vi "Update Device ID.vi"(8 "error in (no error)":errorcluster caption="에러 입력(에러 없음)", 11 "Instrument Manager 입력":refnum<class "Instrument Manager.lvclass">) -> (0 "error out":errorcluster caption="에러 출력", 3 "Instrument Manager 출력":refnum<class "Instrument Manager.lvclass">)   [LabVIEW 2023, in "Instrument Manager.lvclass"]
uses:
  Instrument Manager.lvclass
  Instrument Manager.lvclass/Instrument Manager.ctl
  Module/Turn Table and Mast Control/Class/CO3000/CO3000.lvclass
  Module/Turn Table and Mast Control/Interface Class/Turn Table/Interface - Turn Table.lvclass
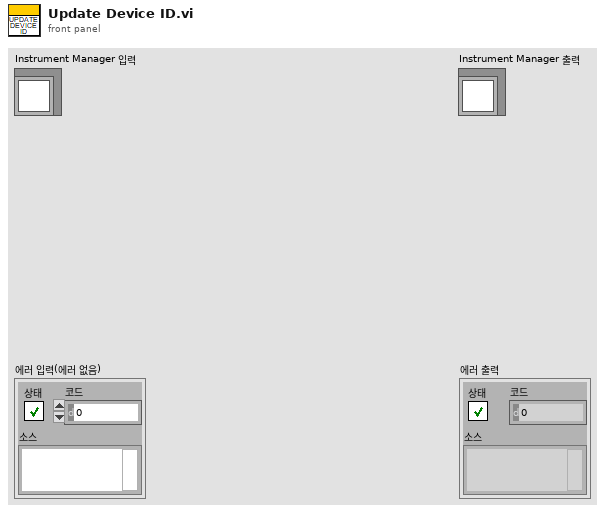
[diagram p1: front panel]
types:
  T1 = cluster{"Anritsu Call Box":refnum<class "Anritsu Call Box.lvclass">, "Spectrum Analyzer":refnum<class "Interface_Spectrum.lvclass">, "RF Switch Box":refnum<class "RF Filter Box.lvclass">, "Turn Table":refnum<class "Interface - Turn Table.lvclass">, "Mast":refnum<class "Interface - Mast.lvclass">, "3D Controller":refnum<class "Interface_3D Controller.lvclass">}
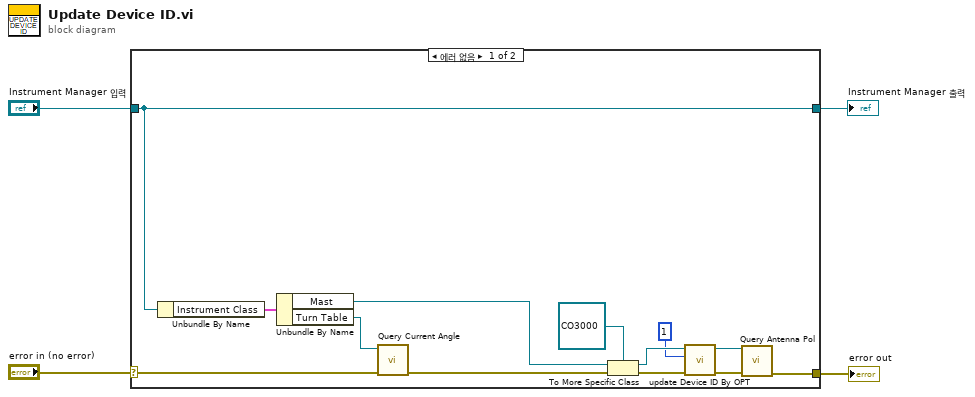
[diagram p0: block diagram]
diagram:
  n1 = case shown="에러 없음" "error in (no error)" {
    selector: "error in (no error)" -> [w16 w19]
    tunnel: [w6 w19] -> w3
    tunnel: [w5 w18] -> w1
    tunnel: "Instrument Manager 입력" -> [w5 w18]
    frame No Error {
      n2 = Unbundle By Name(w5) -> ("Instrument Class"=w17:T1)
      n3 = Unbundle By Name(w17) -> ("Mast"=w12:refnum<class "Interface - Mast.lvclass">, "Turn Table"=w15:refnum<class "Interface - Turn Table.lvclass">)
      n4 = call-dynamic "Query Current Angle.vi"("error in (no error)"=w16, "Interface - Turn Table in"=w15) -> ("error out"=w13:errorcluster)  [unwired: 7 in, 2 out]
      n5 = To More Specific Class(target class=refnum<class "CO3000.lvclass"> refnum ("Turn Table and Mast.lvlib:CO3000.lvclass"), reference=w12, error in=w13) -> (specific class reference=w11:refnum<class "CO3000.lvclass">, error out=w10:errorcluster)
      n6 = call "update Device ID By OPT.vi"("error in (no error)"=w10, "Mast Index"=1, "CO3000 in"=w11) -> ("error out"=w8:errorcluster, "CO3000 out"=w9:refnum<class "CO3000.lvclass">)  [unwired: 5 in, 2 out]
      n7 = call-dynamic "Query Antenna Pol.vi"("error in (no error)"=w8, "CO3000 in"=w9) -> ("error out"=w6:errorcluster)  [unwired: 7 in, 2 out]
    }
    frame Error {
    }
  }
  "error out" <- w3
  "Instrument Manager 출력" <- w1
